vi "GetServerRef.vi"(7 "Connection Configuration":refnum<class "Connection.lvclass">, 8 "error in":errorcluster, 10 "Force Destroy (F)":bool, 11 "Destroy (F)":bool) -> (0 "error out":errorcluster, 2 "Server":refnum<class "Server.lvclass">, 3 "Created":bool, 4 "Connection Config":refnum<class "Connection.lvclass">)   [LabVIEW 2013]
uses:
  source/Server class/Server.lvclass
  <vilib>/LabVIEW Open Source Project/MQTT Connection/MQTT_Connection/Connection/Connection.lvclass
  source/Server class/Server.lvclass/Server.ctl
  <vilib>/LabVIEW Open Source Project/MQTT Connection/MQTT_Base/Base Class/MQTT_Base.lvclass
  <vilib>/LabVIEW Open Source Project/MQTT TCP Connection/MQTT_TCP/Connection/TCPConnection.lvclass
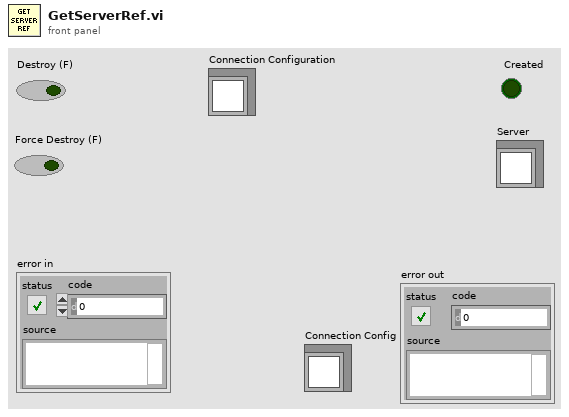
[diagram p1: front panel]
types:
  T1 = typedef "MQTT Server.lvlib/Server.lvclass/Public Events -- cluster.ctl" = cluster{"NbConnections":refnum<user-event>}
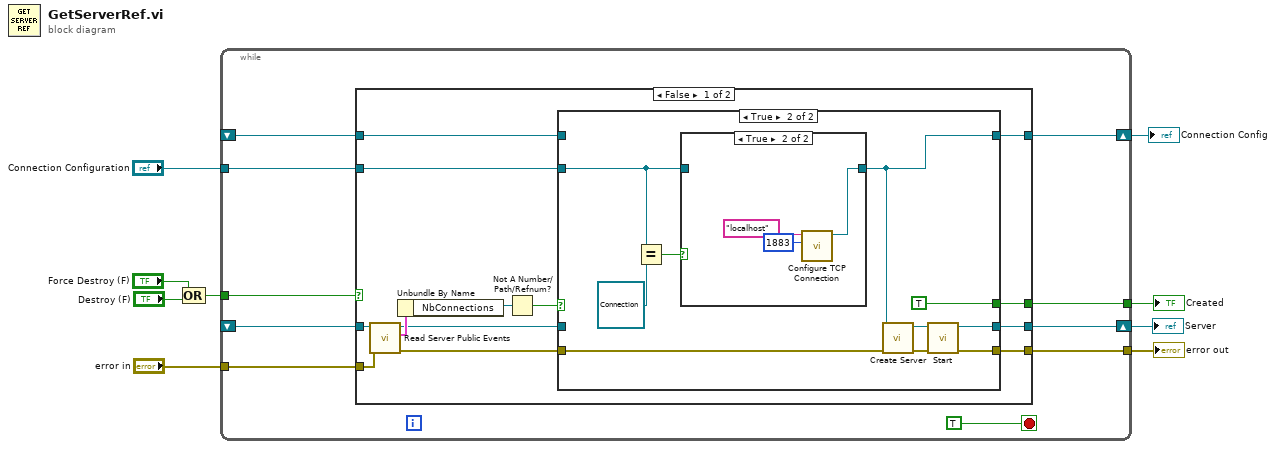
[diagram p0: block diagram]
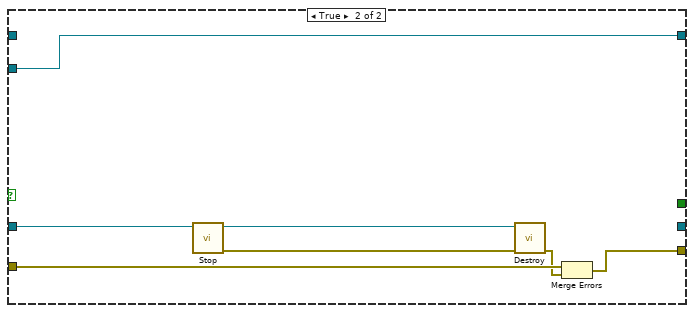
[diagram p4: hidden frame]
diagram:
  n1 = Compound Arithmetic op=OR("Force Destroy (F)", "Destroy (F)") -> (w6:bool)
  n2 = while {
    shift-right: [w18] -> w9
    shift-left: _ -> [w15]
    tunnel: [w17] -> w8
    tunnel: w6 -> [w16]
    tunnel: [w14] -> w7
    tunnel: "error in" -> [w13]
    tunnel: "Connection Configuration" -> [w12]
    shift-right: [w11] -> w2
    shift-left: _ -> [w10]
    stop <- TRUE stop-if-true
    n3 = case shown="False" w16 {
      tunnel: [w32 _] -> w18
      tunnel: [w31 w51] -> w14
      tunnel: [w30 _] -> w17
      tunnel: w15 -> [w29 w54]
      tunnel: w13 -> [w24 w53]
      tunnel: w12 -> [w23 w50]
      tunnel: [w22 w50] -> w11
      tunnel: w10 -> [w21 _]
      frame False {
        n4 = call "Read Server Public Events.vi"("error in (no error)"=w24, "Server in"=w29) -> ("error out"=w25:errorcluster, "MQTT Server.Public Events"=w28:T1, "Server out"=w26:refnum<class "Server.lvclass">)  [unwired: 7 in]
        n5 = Unbundle By Name(w28) -> ("NbConnections"=w27:refnum<user-event>)
        n6 = Not A Number/Path/Refnum?(number/path/refnum=w27) -> (NaN/Path/Refnum?=w20:bool)
        n7 = case shown="True" w20 {
          tunnel: [w35 w45] -> w32
          tunnel: [w34 w44] -> w31
          tunnel: [_ TRUE] -> w30
          tunnel: w26 -> [w35 _]
          tunnel: w25 -> [w34 w42]
          tunnel: w23 -> [_ w38]
          tunnel: [w33 w37] -> w22
          tunnel: w21 -> [w33 _]
          frame False {
          }
          frame True {
            n8 = Equal?(x=w38, y=refnum<class "Connection.lvclass"> refnum ("Connection Configuration")) -> (x = y?=w39:bool)
            n9 = case shown="True" w39 {
              tunnel: w38 -> [w46 _]
              tunnel: [w46 w47] -> w37
              frame False {
              }
              frame True {
                n10 = call <vilib>:"Configure TCP Connection.vi"("remote port (80)"=u16 1883, "address (localhost)"="localhost") -> ("TCPConnection"=w47:refnum<class "TCPConnection.lvclass">)  [unwired: 8 in, 1 out]
              }
            }
            n11 = call "Create Server.vi"("error in (no error)"=w42, "Connection Configuration"=w37) -> ("error out"=w40:errorcluster, "Server"=w41:refnum<class "Server.lvclass">)  [unwired: 8 in]
            n12 = call <vilib>:"Start.vi"("error in (no error)"=w40, "MQTT_Base in"=w41) -> ("error out"=w44:errorcluster, "MQTT_Base out"=w45:refnum<class "Server.lvclass">)  [unwired: 7 in, 1 out]
          }
        }
      }
      frame True {
        n13 = call <vilib>:"Stop.vi"("MQTT_Base in"=w54) -> ("error out"=w55:errorcluster, "MQTT_Base out"=w56:refnum<class "Server.lvclass">)  [unwired: 8 in, 1 out]
        n14 = call <vilib>:"Destroy.vi"("error in (no error)"=w55, "MQTT_Base in"=w56) -> ("error out"=w52:errorcluster)  [unwired: 8 in, 1 out]
        n15 = Merge Errors(w53, w52) -> (w51:errorcluster)
      }
    }
  }
  "Server" <- w9
  "Created" <- w8
  "error out" <- w7
  "Connection Config" <- w2
